vi "Main.vi"   [LabVIEW 2019]
doc: "Main interface to Dataflow DJ.\n\n<b>Execution System:</b> User Interface"
uses:
  Libraries/User Interface/Sub Panels Cluster.ctl
  Libraries/Track Info/Track Info FGV Enum.ctl
  Libraries/Audio Output/Audio Output Queue Type.ctl
  Libraries/Config File/Config Cluster.ctl
  Libraries/Track Info/Track Info.ctl
  <vilib>/Analysis/1siggen.llb/Ramp Pattern by Samples.vi
  Packed Libraries/Globals.lvlibp/Constants.vi
  <vilib>/Platform/TimedLoop/scheduler/LVUserAPI/_suppVIs/Create_SoftwareTrigger_TSource.vi
  Plugin Interfaces/Controller Interface/Controller Interface.lvlibp/Controller Interface Class/Controller Interface.lvclass
  Libraries/Audio Engine/Audio Engine.lvlib
  Libraries/Audio Output/Audio Output.lvlib
  Packed Libraries/Globals.lvlibp
  Libraries/User Interface/User Interface.lvlib
  Libraries/Config File/Config File.lvlib
  Libraries/Track Info/Track Info.lvlib
  <vilib>/Analysis/NI_AALBase.lvlib
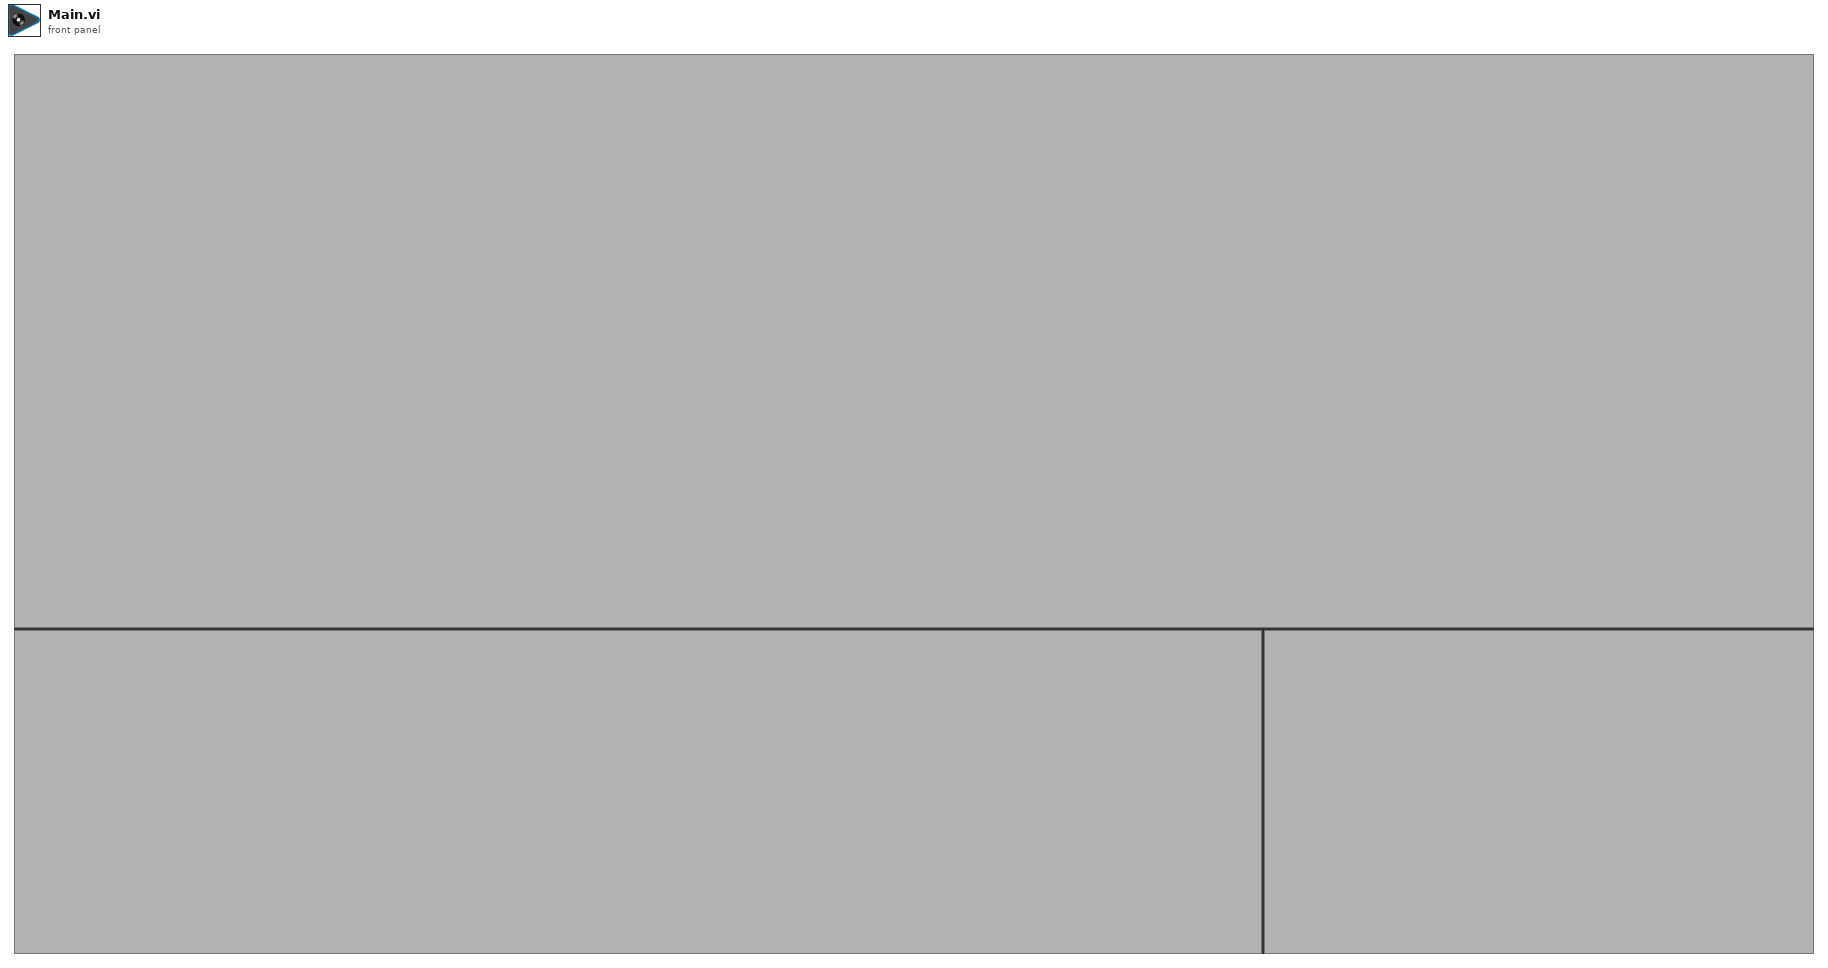
[diagram p1: front panel]
types:
  T1 = typedef "User Interface.lvlib/Sub Panels Cluster.ctl" = cluster{"DJ Interface":refnum<vi>, "File Browser":refnum<vi>, "Audio Config":refnum<vi>}
  T2 = typedef "Track Info.lvlib/Track Info FGV Enum.ctl" = enum16{"Init", "Update Track", "Update Multiple Tracks", "Get Track", "Get Multiple Tracks"}
  T3 = typedef "Audio Output.lvlib/Audio Output Queue Type.ctl" = cluster{"Master":waveform(i16)[], "Headphones":waveform(i16)[], "Start Time":dbl}
  T4 = typedef "Config File.lvlib/Config Cluster.ctl" = cluster{"Track Info":T5[]}
  T5 = typedef "Track Info.lvlib/Track Info.ctl" = cluster{"Path":path, "Length (Samples)":i32, "Channels":i32, "Sample Rate (Hz)":i32, "BPM":dbl, "Cue Points (Samples)":i32[]}
  T6 = enum32{"invalid app kind", "Development System", "Run Time System", "Student Edition", "Embedded LabVIEW", "Evaluation", "Custom"}
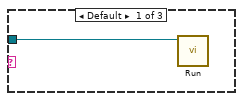
[diagram p2: hidden frame]
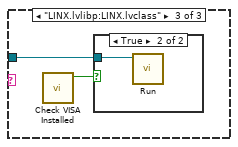
[diagram p4: hidden frame]
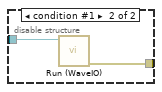
[diagram p6: hidden frame]
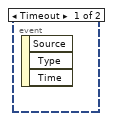
[diagram p7: hidden frame]
diagram:
  w13 = FALSE  # Shutdown
  # "#TODO\nOffload this checking logic to the class itself"
  # "Load WaveIO VIs programmatically\n\nif waveio.dll exists, then dynamically call VIs in waveio.llb\nif it doesn't exist, fall back to lvsound2.dll\n\nshould also address this issue"
  # "Startup order required\nAudio Processing\n- Setup message queues for all control messages from UI and hardware\n- Begin generating output data\nAutio Output\n- Setup message queue from audio config UI panel\nUser Interface (DJ Interface)\n- Setup message queue to receive UI changes\n- Scan all UI elements and send values and limits to Audio Processing\nHardware Controller\n- Setup hardware and read current IO state\n- Send IO state to Audio Processing, which will then relay changes back to UI\n\n#TODO Use named Notifiers to wait for each component to start up"
  # "EXECUTION SYSTEMS\n\nAudio Processing.Run.vi    Standard\nAudio Output.Run.vi    Instrument I/O\nMain.vi    User Interface\nUser Interface.DJ Interface.vi    User Interface\nUser Interface.File Browser.vi    User Interface\nUser Interface.Audio Config.vi    User Interface\nHardware Control.DAQmx Run.vi    Data Acquisition\nAudio File Input.Load Async.vi    Other 1"
  # "Dataflow DJ - A live DJ mixing application written entirely in LabVIEW.\n    Copyright (C) 2019  Dataflow G\n    \n    This program is free software: you can redistribute it and/or modify\n    it under the terms of the GNU General Public License as published by\n    the Free Software Foundation, either version 3 of the License, or\n    (at your option) any later version.\n\n    This program is distributed in the hope that it will be useful,\n    but WITHOUT ANY WARRANTY; without even the implied warranty of\n    MERCHANTABILITY or FITNESS FOR A PARTICULAR PURPOSE.  See the\n    GNU General Public License for more details.\n\n    You should have received a copy of the GNU General Public License\n    along with this program.  If not, see <https://www.gnu.org/licenses/>.\n\nContact:\n    GitHub - https://github.com/dataflowg\n    Twitter - @Dataflow_G"
  # "If the WaveIO library is installed in external\\waveio_108, set WaveIO to TRUE in the Project's conditional disable symbols to use it here. \n\n#TODO\nAutomatically discover if WaveIO is available for development, maybe with a script or something."
  # "This is the main audio queue between the audio processing loop and audio output loop. It's a single element queue (SEQ) which contains the next block of audio data to be sent to both the master and headphone outputs. The block size is always Buffer Size (see global constant). Using a SEQ means the audio processing loop timing can be slaved to the audio output loop timing."
  # "Down, down, down. Would the fall NEVER come to an end!"
  n1 = flat-sequence {
    tunnel: [w32] -> w5
    tunnel: [w29] -> w4
    frame #0 {
      # "Initialise Zero Buffer. This is sent to the soundcard when a track isn't loaded, is paused, or the headphone cue is disabled."
      n2 = global read "Constants.vi" "Buffer Size"() -> (w18:i32)
      n3 = global read "Constants.vi" "Channels"() -> (w19:i32)
      n4 = call "Track Info FGV.vi"("Track Info FGV Enum"=Track_Info_FGV_Enum."Init") -> ("error out"=w24:errorcluster)  [unwired: 7 in, 3 out]
      n5 = call-poly <vilib>:"Ramp Pattern.vi"("start"=0.0, "end"=1.0, "samples"=w18) -> ("Ramp Pattern"=w17:dbl[])  [unwired: 7 in, 1 out]
      n6 = call "Load Config.vi"("error in (no error)"=w24) -> ("Config"=w22:T4)  [unwired: 9 in, 1 out]
      n7 = Initialize Array(0.0, w19, w18) -> (w28:dbl[][])
      n8 = Unbundle By Name(w22) -> ("Track Info"=w26:T5[])
      n9 = Reverse 1D Array(array=w17) -> (reversed array=w16:dbl[])
      n10 = global write "Constants.vi" "Zero Buffer"(w28) -> ()
      n11 = global write "Constants.vi" "Ramp (Fade In)"(w17) -> ()
      n12 = global write "Constants.vi" "Ramp (Fade Out)"(w16) -> ()
      n13 = call "Track Info FGV.vi"("Track Info FGV Enum"=Track_Info_FGV_Enum."Update Multiple Tracks", "Multiple Track Info In"=w26) -> ()  [unwired: 6 in, 4 out]
    }
    frame #1 {
      n14 = call-poly <vilib>:"Create Timing Source.vi"("trigger ID"=u8 0) -> ("timing source name"=w29:string)  [unwired: 9 in, 1 out]
      n15 = Obtain Queue(max queue size (-1, unlimited)=1, name (unnamed)="Audio", element data type=T3 {"Master"=[], "Headphones"=[], "Start Time"=0.0}) -> (queue out=w32:refnum<queue>)  [unwired: 2 in, 2 out]
    }
  }
  n16 = control-ref of="DJ Interface Sub Panel"() -> (w11:refnum<vi>)
  n17 = control-ref of="File Browser Sub Panel"() -> (w10:refnum<vi>)
  n18 = control-ref of="Audio Config Sub Panel"() -> (w9:refnum<vi>)
  n19 = Bundle By Name(cluster=T1 {"DJ Interface"=refnum, "File Browser"=refnum, "Audio Config"=refnum} ("Sub Panels"), "DJ Interface"=w11, "File Browser"=w10, "Audio Config"=w9) -> (w8:T1)
  n20 = control-ref of="This VI"() -> (w7:refnum<vi>)
  n21 = Create User Event(user event datatype=w13) -> (user event=w3:refnum<user-event>, error out=w6:errorcluster)  [unwired: 1 in]
  n22 = call "Insert Sub Panels.vi"("error in (no error)"=w6, "Shutdown Event"=w3, "Sub Panels"=w8, "Owning VI"=w7) -> ()  [unwired: 7 in, 1 out]
  n23 = while {
    tunnel: w3 -> [w37]
    tunnel: w5 -> [w36]
    tunnel: w4 -> [w35]
    stop <- w38 stop-if-true
    n24 = event shown="[1] Panel Close?" {
      selector: _ -> [_ _]
      dyn-events: _ -> [_ _]
      timeout: _ -> [_ _]
      tunnel: [_ TRUE] -> w38
      tunnel: w37 -> [_ w52]
      tunnel: w36 -> [_ w46]
      tunnel: w35 -> [_ w39]
      event Timeout {
        n25 = event-data() -> ()  [unwired: 1 in, 3 out]
      }
      event Panel Close? {
        # "Write track info and config to disk on shutdown"
        # "Only close the panel if running under the run-time engine."
        n26 = event-data() -> ()  [unwired: 1 in, 4 out]
        n27 = Generate User Event(user event=w52, event data cluster=TRUE ("event data")) -> (user event out=w50:refnum<user-event>, error out=w49:errorcluster)  [unwired: 2 in]
        n28 = call "Track Info FGV.vi"("Track Info FGV Enum"=Track_Info_FGV_Enum."Get Multiple Tracks") -> ("Multiple Track Info Out"=w44:T5[])  [unwired: 7 in, 3 out]
        n29 = Destroy User Event(user event=w50, error in=w49) -> (error out=w45:errorcluster)
        n30 = Bundle By Name(cluster=T4 {"Track Info"=[]} ("Config"), "Track Info"=w44) -> (w43:T4)
        n31 = call "Save Config.vi"("Config"=w43) -> ()  [unwired: 10 in, 1 out]
        n32 = Release Queue(queue=w46, force destroy? (F)=TRUE, error in (no error)=w45) -> (error out=w40:errorcluster)  [unwired: 2 out]
        n33 = call <vilib>:"Clear Timing Source.vi"("error in (no error)"=w40, "name"=w39) -> ()  [unwired: 8 in, 2 out]
        n34 = property class="App"() -> ("App.Kind"=w55:T6)  [unwired: 2 in, 2 out]
        n35 = Not Equal?(x=w55, y=T6."Run Time System") -> (x != y?=w48:bool)
        n36 = event-data("Discard?"=w48) -> ()  [unwired: 1 in, 1 out]
      }
    }
  }
  n37 = call "Load Controller Plugins.vi"("Shutdown Event"=w3) -> ("Controller Plugins"=w2:refnum<class "Controller Interface.lvclass">[])  [unwired: 10 in]
  n38 = Array Size(array=w2) -> (size(s)=w1:i32)
  n39 = disable-structure shown="Default" {
    disable-tunnel: w5 -> [w57 w59]
    disable-tunnel: [w56 w58] -> w15
    frame condition #0 (active) {
      n40 = call "Run (lvsound2).vi"("Audio Output Queue"=w57) -> ("error out"=w56:errorcluster)  [unwired: 10 in]
    }
    frame condition #1 {
      n41 = call "Run (WaveIO).vi"("Audio Output Queue"=w59) -> ("error out"=w58:errorcluster)  [unwired: 10 in]
    }
  }
  n42 = for {
    tunnel: w2 -> [w60] mode=indexing
    workers-P: w1 -> [_]
    n43 = call <vilib>:"Get LV Class Name.vi"("object"=w60) -> ("class name"=w61:string)  [unwired: 9 in, 1 out]
    n44 = case shown="\"DAQmx.lvlibp:DAQmx.lvclass\"" w61 {
      tunnel: w60 -> [w62 w64 w67]
      frame Default {
        n45 = call-dynamic "Run.vi"("Controller Interface in"=w62) -> ()  [unwired: 9 in, 2 out]
      }
      frame "DAQmx.lvlibp:DAQmx.lvclass" {
        n46 = call "Check DAQmx Installed.vi"() -> ("DAQmx Installed?"=w63:bool)  [unwired: 11 in]
        n47 = case shown="True" w63 {
          tunnel: w64 -> [_ w65]
          frame False {
          }
          frame True {
            n48 = call-dynamic "Run.vi"("Controller Interface in"=w65) -> ()  [unwired: 9 in, 2 out]
          }
        }
      }
      frame "LINX.lvlibp:LINX.lvclass" {
        n49 = call "Check VISA Installed.vi"() -> ("VISA Installed?"=w66:bool)  [unwired: 11 in]
        n50 = case shown="True" w66 {
          tunnel: w67 -> [_ w68]
          frame False {
          }
          frame True {
            n51 = call-dynamic "Run.vi"("Controller Interface in"=w68) -> ()  [unwired: 9 in, 2 out]
          }
        }
      }
    }
  }
  n52 = call "Run.vi"("Timing Source"=w4, "Audio Output Queue"=w5) -> ()  [unwired: 9 in, 1 out]
  n53 = call <vilib>:"General Error Handler.vi"("error in (no error)"=w15) -> ("error out"=w14:errorcluster)  [unwired: 10 in, 4 out]
  n54 = call ".vi"("error in (no escape)"=w14) -> ()
